vi "Frontpanel Scratchpad.vi"() -> ()   [LabVIEW 2019]
uses:
  Typedefs/KH Mode-enum.ctl
  Control Experiment.lvclass
  <userlib>/LevyLab/Krohn Hite 7008/KH7008/typedefs/Input--Enum.ctl
  <userlib>/LevyLab/Krohn Hite 7008/KH7008/KH7008.lvlib
  <userlib>/LevyLab/Krohn Hite 7008/KH7008/typedefs/gain--enum.ctl
  <userlib>/LevyLab/Krohn Hite 7008/KH7008/typedefs/shunt--enum.ctl
panel:
  in  "KH":T4 {"KH #" items=["A 1", "A 2", "A 3", "A 4", "A 5", "A 6", "A 7", "A 8"]}
  in  "System Array":T6(array[cluster]) {"Ring" items=["V", "U", "n.c."]}
  in  "Channel Setting":T7(array[cluster]) {"channel" min=1 max=8 step=1}
  in  "Lockin":T8 {"Label" items=["", "I+", "I-", "V1+", "V1-", "V2+", "V2-", "V3+", "V3-", "V4+", "V4-", "dV1", "dV2", "dV3", "Vsg", "Vbg", "Vtg"]}
  # "KH"
  # "electrode"
  # "Symbol"
  # "label"
  # "KH config"
  # "KH"
  # "gain"
  # "input"
  # "shunt"
  # "coupling"
  # "filter"
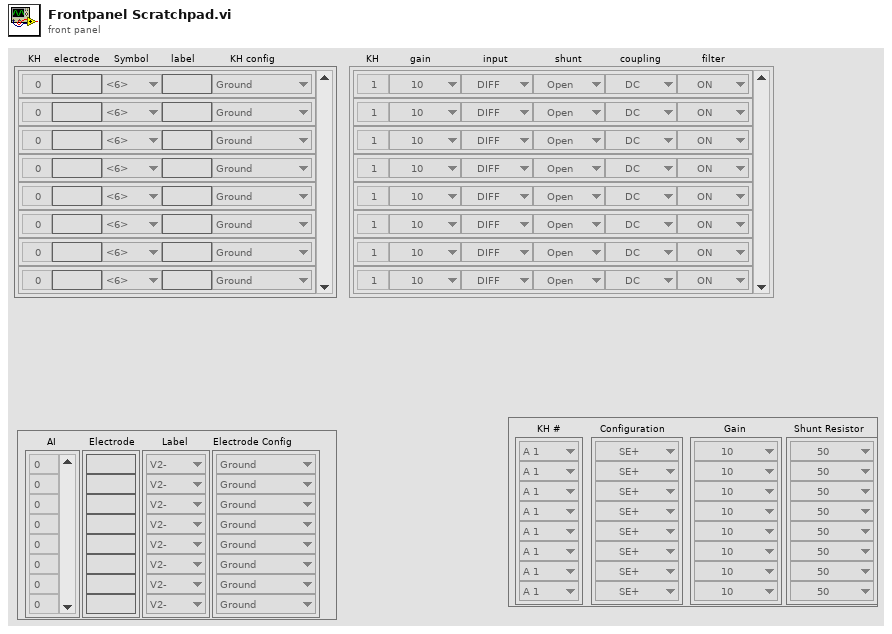
[diagram p1: front panel]
types:
  T1 = typedef "KH7008.lvlib/Input--Enum.ctl" = enum16{"OFF", "SE+", "SE-", "DIFF"}
  T2 = typedef "KH7008.lvlib/gain--enum.ctl" = enum16{"1", "10", "100", "1000"}
  T3 = typedef "KH7008.lvlib/shunt--enum.ctl" = enum16{"Open", "50", "500", "5k", "50k", "10M"}
  T4 = cluster{"KH #":u16[], "KH Configuration":T1[], "KH Gain":T2[], "KH Shunt Resistor":T3[]}
  T5 = typedef "Control Experiment.lvclass/KH Mode-enum.ctl" = enum16{"Ground", "Current", "Voltage (SE)", "Voltage (Diff)", "Gate"}
  T6 = cluster{"Numeric":u32, "electrode":string, "Ring":u16, "label":string, "Enum":T5}[]
  T7 = cluster{"channel":u16, "gain":enum16{"1", "10", "100", "1000"}, "input":enum16{"OFF", "SE+", "SE-", "DIFF"}, "shunt":enum16{"Open", "50", "500", "5k", "50k", "10M"}, "couple":enum16{"AC", "DC"}, "filter":enum16{"OFF", "ON"}}[]
  T8 = cluster{"AI":u32[], "Electrode":string[], "Label":u16[], "Electrode Config":T5[]}
  T9 = cluster{"Numeric":u32, "electrode":string, "Ring":u16, "label":string, "Enum":T5}
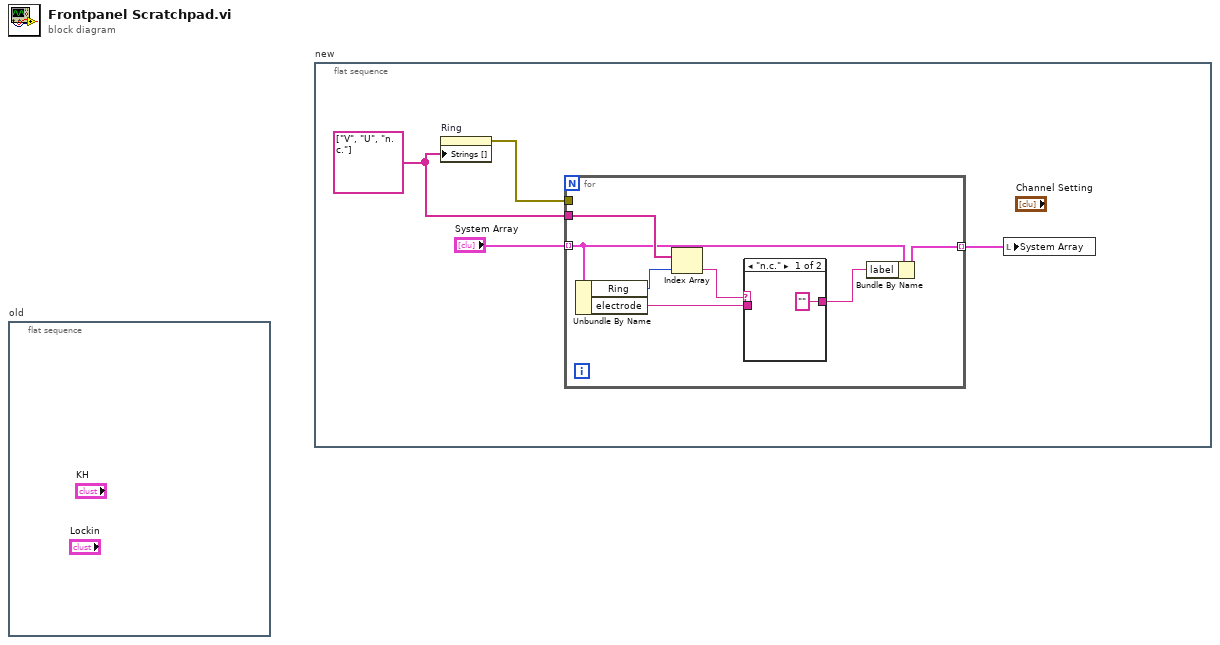
[diagram p0: block diagram]
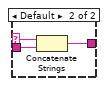
[diagram p2: hidden frame]
diagram:
  n1 = flat-sequence "old" {
    frame #0 {
    }
  }
  n2 = flat-sequence "new" {
    frame #0 {
      w2 = string[] ["V", "U", "n.c."] ("Strings []")
      n3 = property on="Ring" class="Ring (strict)"("Strings []"=w2) -> (error out=w4:errorcluster)  [unwired: 2 in, 1 out]
      n4 = for {
        tunnel: w4 -> [_]
        tunnel: "System Array" -> [w9] mode=indexing
        tunnel: w2 -> [w10]
        tunnel: [w5] -> w1 mode=indexing
        n5 = Unbundle By Name(w9) -> ("Ring"=w11:u16, "electrode"=w7:string)
        n6 = Index Array(array=w10, index=w11) -> (element=w8:string)
        n7 = case shown="\"n.c.\"" w8 {
          selector: w8 -> [_ w15]
          tunnel: w7 -> [_ w14]
          tunnel: ["" w13] -> w6
          frame "n.c." {
          }
          frame Default {
            n8 = Concatenate Strings(w15, w14) -> (w13:string)
          }
        }
        n9 = Bundle By Name(cluster=w9, "label"=w6) -> (w5:T9)
      }
      n10 = local write "System Array"(w1) -> ()
    }
  }
